vi "Variable globale compteurs.vi"() -> ()   [LabVIEW 2022 SP3]
panel:
  out "data+debit compteurs":string[][](array[string])
  out "Temps débit":u16
  in  "Tache Compteurs":T1 {"Init compteurs" format="%.2f"}
  out "data compteurs":string[](array[string])
  in  "COMPTEURS":bool
  # "Compteurs GN2"
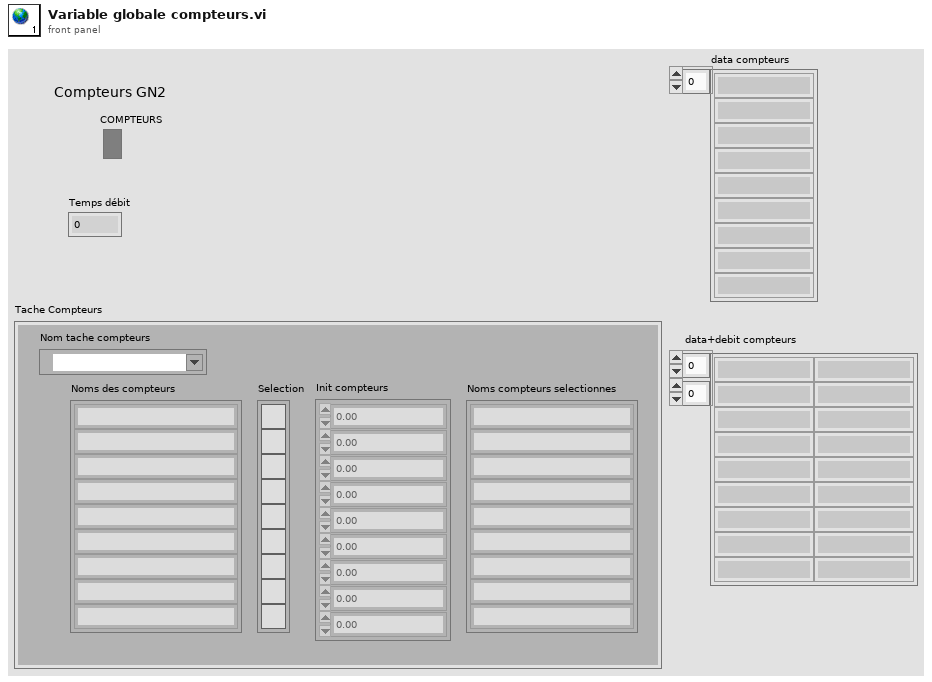
[diagram p1: front panel]
types:
  T1 = cluster{"Nom tache compteurs":refnum<k21>, "Noms des compteurs":string[], "Selection":bool[], "Init compteurs":dbl[], "Noms compteurs selectionnes":string[]}
diagram:
